vi "RFH-convert-general-folder.vi"(5 "Destination Folder":path, 7 "folder path":path, 8 "error in (no error)":errorcluster) -> (0 "error out":errorcluster, 1 "Data":T1, 2 "converted file path":path)   [LabVIEW 2020, in "RFH-Reflection_File_Handler.lvlib"]
doc: "Converts every file in a folder to the common format and saves it in the destination folder. Returns the last data and its path."
uses:
  RFH-Reflection_File_Handler.lvlib
  RFH-common_data_format.ctl
panel:
  in  "Use tamplate?":bool
  in  "New Name":string
  in  "Replace Name":string
  in  "X template":path=path "C:/projects/Universitet/Master/data/Ideal data/Compare/PB1-water.s2p"
  in  "Max Frequency":dbl=6000000000.0 format="%#_6p"
  in  "min Frequency":dbl=300000000.0 format="%#_6p"
  in  "sim":bool
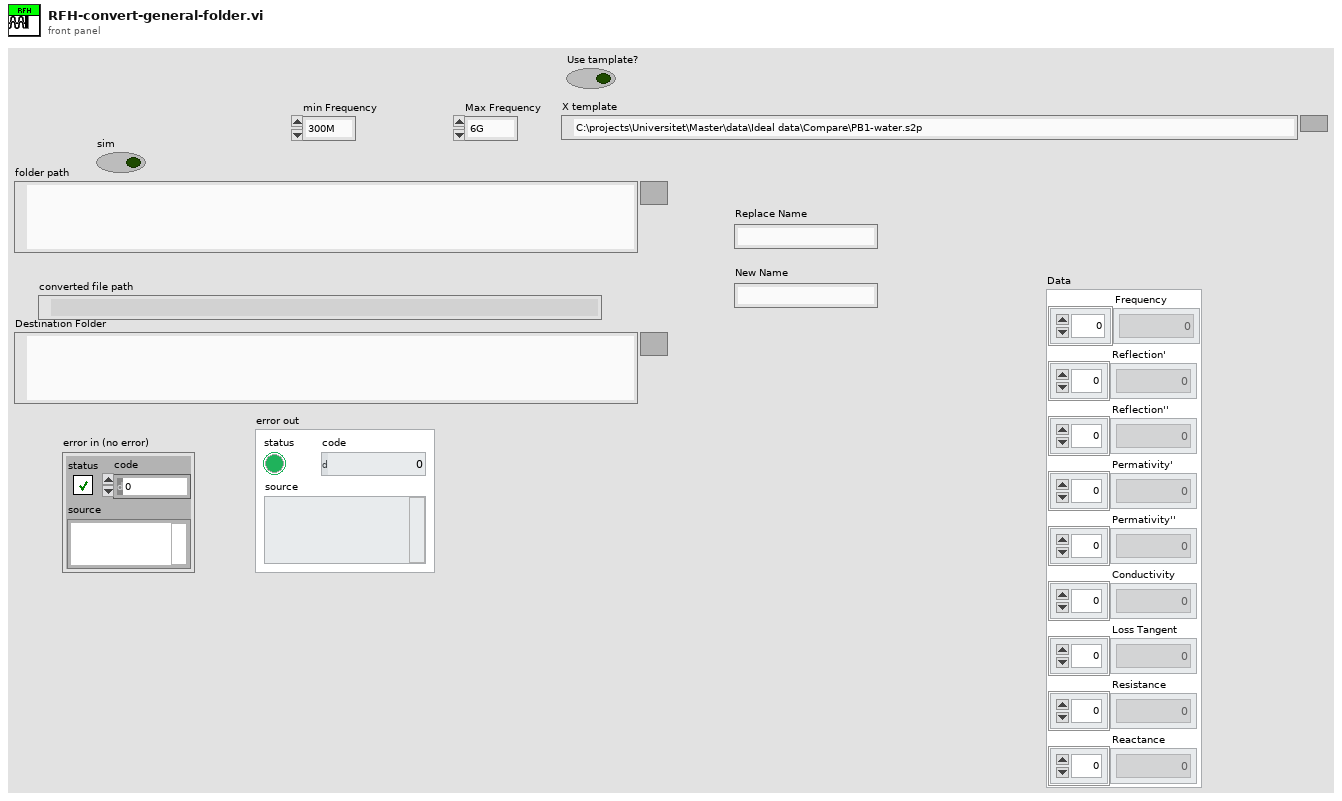
[diagram p1: front panel]
types:
  T1 = typedef "RFH-Reflection_File_Handler.lvlib/RFH-common_data_format.ctl" = cluster{"Frequency":dbl[], "Reflection'":dbl[], "Reflection''":dbl[], "Permativity'":dbl[], "Permativity''":dbl[], "Conductivity":dbl[], "Loss Tangent":dbl[], "Resistance":dbl[], "Reactance":dbl[]}
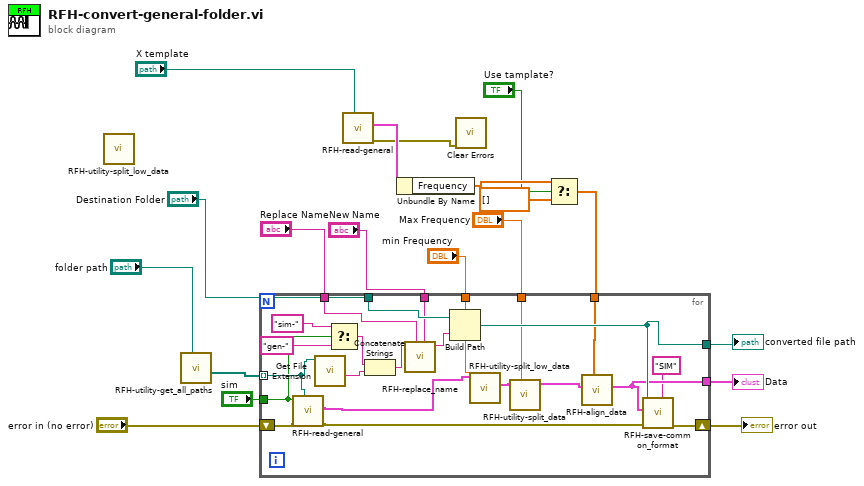
[diagram p0: block diagram]
diagram:
  n1 = call "RFH-utility-split_low_data.vi"() -> ()  [unwired: 11 in, 1 out]
  n2 = call "RFH-utility-get_all_paths.vi"("Folder Path"="folder path") -> ("All Files in Dir"=w12:path[])  [unwired: 7 in, 3 out]
  n3 = call "RFH-read-general.vi"("file path (dialog if empty)"="X template") -> ("error out"=w7:errorcluster, "Common Format"=w8:T1)  [unwired: 9 in]
  n4 = Unbundle By Name(w8) -> ("Frequency"=w4:dbl[])
  n5 = call <vilib>:"Clear Errors.vi"("error in (no error)"=w7) -> ()  [unwired: 5 in, 2 out]
  n6 = Select(t=w4, s="Use tamplate?", f=dbl[] []) -> (s? t:f=w2:dbl[])
  n7 = for {
    tunnel: w2 -> [w35]
    tunnel: "sim" -> [w31]
    tunnel: [w32] -> w14
    shift-right: [w39] -> w17
    shift-left: "error in (no error)" -> [w38]
    tunnel: w12 -> [w36] mode=indexing
    tunnel: "Destination Folder" -> [w40]
    tunnel: [w41] -> w19
    tunnel: "min Frequency" -> [w21]
    tunnel: "Max Frequency" -> [w33]
    tunnel: "Replace Name" -> [w25]
    tunnel: "New Name" -> [w24]
    n8 = call "RFH-read-general.vi"("file path (dialog if empty)"=w36, "error in"=w38, "sim"=w31) -> ("error out"=w37:errorcluster, "Common Format"=w22:T1)  [unwired: 7 in]
    n9 = call <vilib>:"Get File Extension.vi"("file"=w36) -> ("filename without extension"=w42:string)  [unwired: 6 in, 4 out]
    n10 = Select(t="sim-", s=w31, f="gen-" ("string")) -> (s? t:f=w29:string)
    n11 = Concatenate Strings(w29, w42) -> (w27:string)
    n12 = call "RFH-replace_name.vi"("New name"=w24, "replace"=w25, "Filename in"=w27) -> ("Filename out"=w26:string)  [unwired: 8 in]
    n13 = Build Path(base path=w40, name or relative path=w26) -> (appended path=w41:path)
    n14 = call "RFH-utility-split_low_data.vi"("Frequency"=w21, "Common Format"=w22) -> ("After"=w23:T1)  [unwired: 9 in]
    n15 = call "RFH-utility-split_data.vi"("Frequency"=w33, "Common Format"=w23) -> ("Before"=w34:T1)  [unwired: 8 in, 1 out]
    n16 = call "RFH-align_data.vi"("Xi"=w35, "Common Format"=w34) -> ("Common Format alligned"=w32:T1)  [unwired: 9 in]
    n17 = call "RFH-save-common_format.vi"("source"="SIM", "file path (use dialog)"=w41, "error in (no error)"=w37, "Common Format"=w32) -> ("error out"=w39:errorcluster)  [unwired: 7 in]
  }
  "error out" <- w17
  "converted file path" <- w19
  "Data" <- w14
